vi "Set CD Storage Library Loader Ref.vi"(10 "CDS Loader Ref":refnum<vi>, 11 "DMA Channel Testing in":refnum<class "FPGA Addon DMA Channel Unit Tests.lvclass">) -> (3 "DMA Channel Testing out":refnum<class "FPGA Addon DMA Channel Unit Tests.lvclass">)   [LabVIEW 2020, in "FPGA Addon DMA Channel Unit Tests.lvclass"]
uses:
  FPGA Addon DMA Channel Unit Tests.lvclass
  FPGA Addon DMA Channel Unit Tests.lvclass/FPGA Addon DMA Channel Unit Tests.ctl
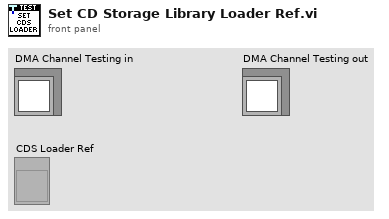
[diagram p1: front panel]
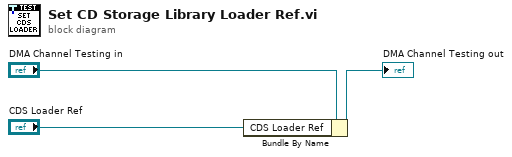
[diagram p0: block diagram]
diagram:
  n1 = Bundle By Name(cluster="DMA Channel Testing in", "CDS Loader Ref"="CDS Loader Ref") -> (→"DMA Channel Testing out":refnum<class "FPGA Addon DMA Channel Unit Tests.lvclass">)
